vi "RT Driver VI.vi"(6 "Device Clock":string, 9 "Device Inputs FIFO":refnum<k33>, 10 "Device Outputs FIFO":refnum<k33>, 11 "Device Reference":T1 format="%.0x") -> ()   [LabVIEW 2025, in "Keithley-DAQ6510 Engine.lvlib"]
uses:
  Keithley-DAQ6510 Engine.lvlib
  <vilib>/NI VeriStand/Custom Device API/Custom Device Item Ref.ctl
  <vilib>/NI VeriStand/Custom Device API/Custom Device Channel Type.ctl
  RT_ctrl.ctl
  <vilib>/NI VeriStand/Custom Device API/Message Response (String).ctl
  <vilib>/NI VeriStand/Custom Device API/Message Response (Byte Array).ctl
  System Explorer/Sys_DAQ_Global.vi
  <vilib>/NI VeriStand/Custom Device API/Get Item Property (Variant).vi
  <vilib>/NI VeriStand/Custom Device API/Get Item Property (String).vi
  <vilib>/NI VeriStand/Custom Device API/Custom Device API.lvlib
  <vilib>/NI VeriStand/Custom Device Tools/Custom Device Utility Library/Custom Device Utility Library.lvlib
  System Explorer/Keithley-DAQ6510 System Explorer.lvlib
  <instrlib>/Keithley DMM6500 DAQ6500 Series/Keithley DMM6500 DAQ6500 Series.lvlib
panel:
  in  "Initialization Status Notifier":refnum<notifier>
  in  "Status Notifier":refnum<notifier>
  # "Custom Device Template\nv1.0"
  # "Use this template as a starting point for creating a custom device code module. The input controls shown here are specially named controls that the system will use to provide the device loop with data. The controls are not required for the device loop to run. For instance, if the device doesn't produce any output data, then you don't need the Device Outputs FIFO control. If you do use these controls, however, they need to have these exact names to be functional."
  # "The optional status notifier element is used to notify the RT engine of the last state of the custom device, and to indicate the device has completed execution. If this control is not used, a default No Error value is returned to the system when the device finishes execution.\n\nNote: This error state is not checked until the system shuts down. Use an output status channel to send more immediate status values to the system."
  # "This optional input can be used to send the VeriStand Engine the final status of the custom device initalization process. If this control exists on the custom device front panel, the VeriStand Engine will wait for a status update before starting up. If the custom device reports an error, that will abort the execution of the current configuration in the VeriStand Engine.\n\nThis control can be deleted if the custom device does not need to send the initialization status update."
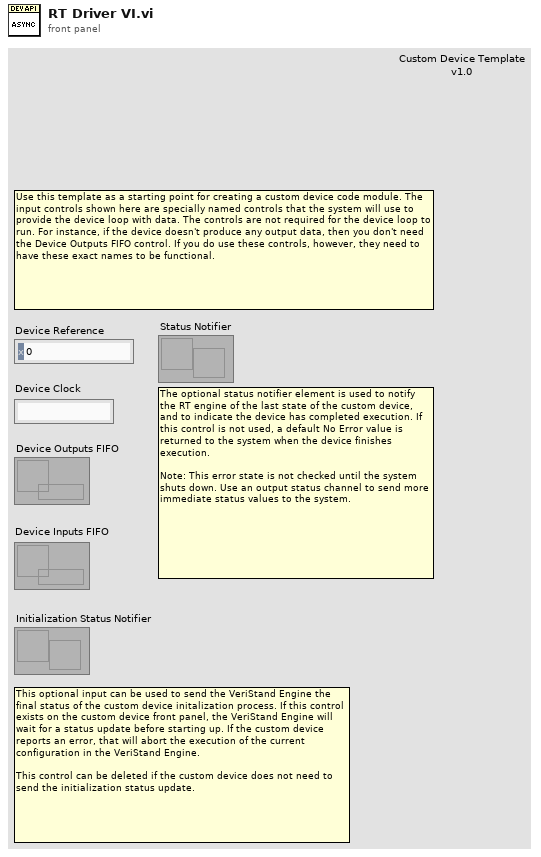
[diagram p1: front panel]
types:
  T1 = typedef "Custom Device API.lvlib/Custom Device Item Ref.ctl" = u64
  T2 = cluster{"Baud Rate":u32, "Flow Control":u16, "Parity":u16, "Stop Bits":u16, "Data Bits":u16}
  T3 = typedef "Keithley-DAQ6510 Engine.lvlib/RT_ctrl.ctl" = cluster{"Device Outputs FIFO":refnum<k33>, "Device Inputs FIFO":refnum<k33>, "Function":i32, "Pseudo Card":i32, "Slot":i32, "Channel_list":string, "Auto/Man":bool, "Manual Range":dbl, "VISA ":refnum<visa-resource-name>}
  T4 = typedef "Custom Device API.lvlib/Custom Device Channel Type.ctl" = enum16{"Input", "Output"}
  T5 = typedef "Custom Device API.lvlib/Custom Device Engine Event Ref.ctl" = refnum<event-registration>
  T6 = typedef "Custom Device API.lvlib/Message Response (String).ctl" = cluster{"Response":string, "Error":errorcluster}
  T7 = typedef "Custom Device API.lvlib/Message Response (Byte Array).ctl" = cluster{"Response":u8[], "Error":errorcluster}
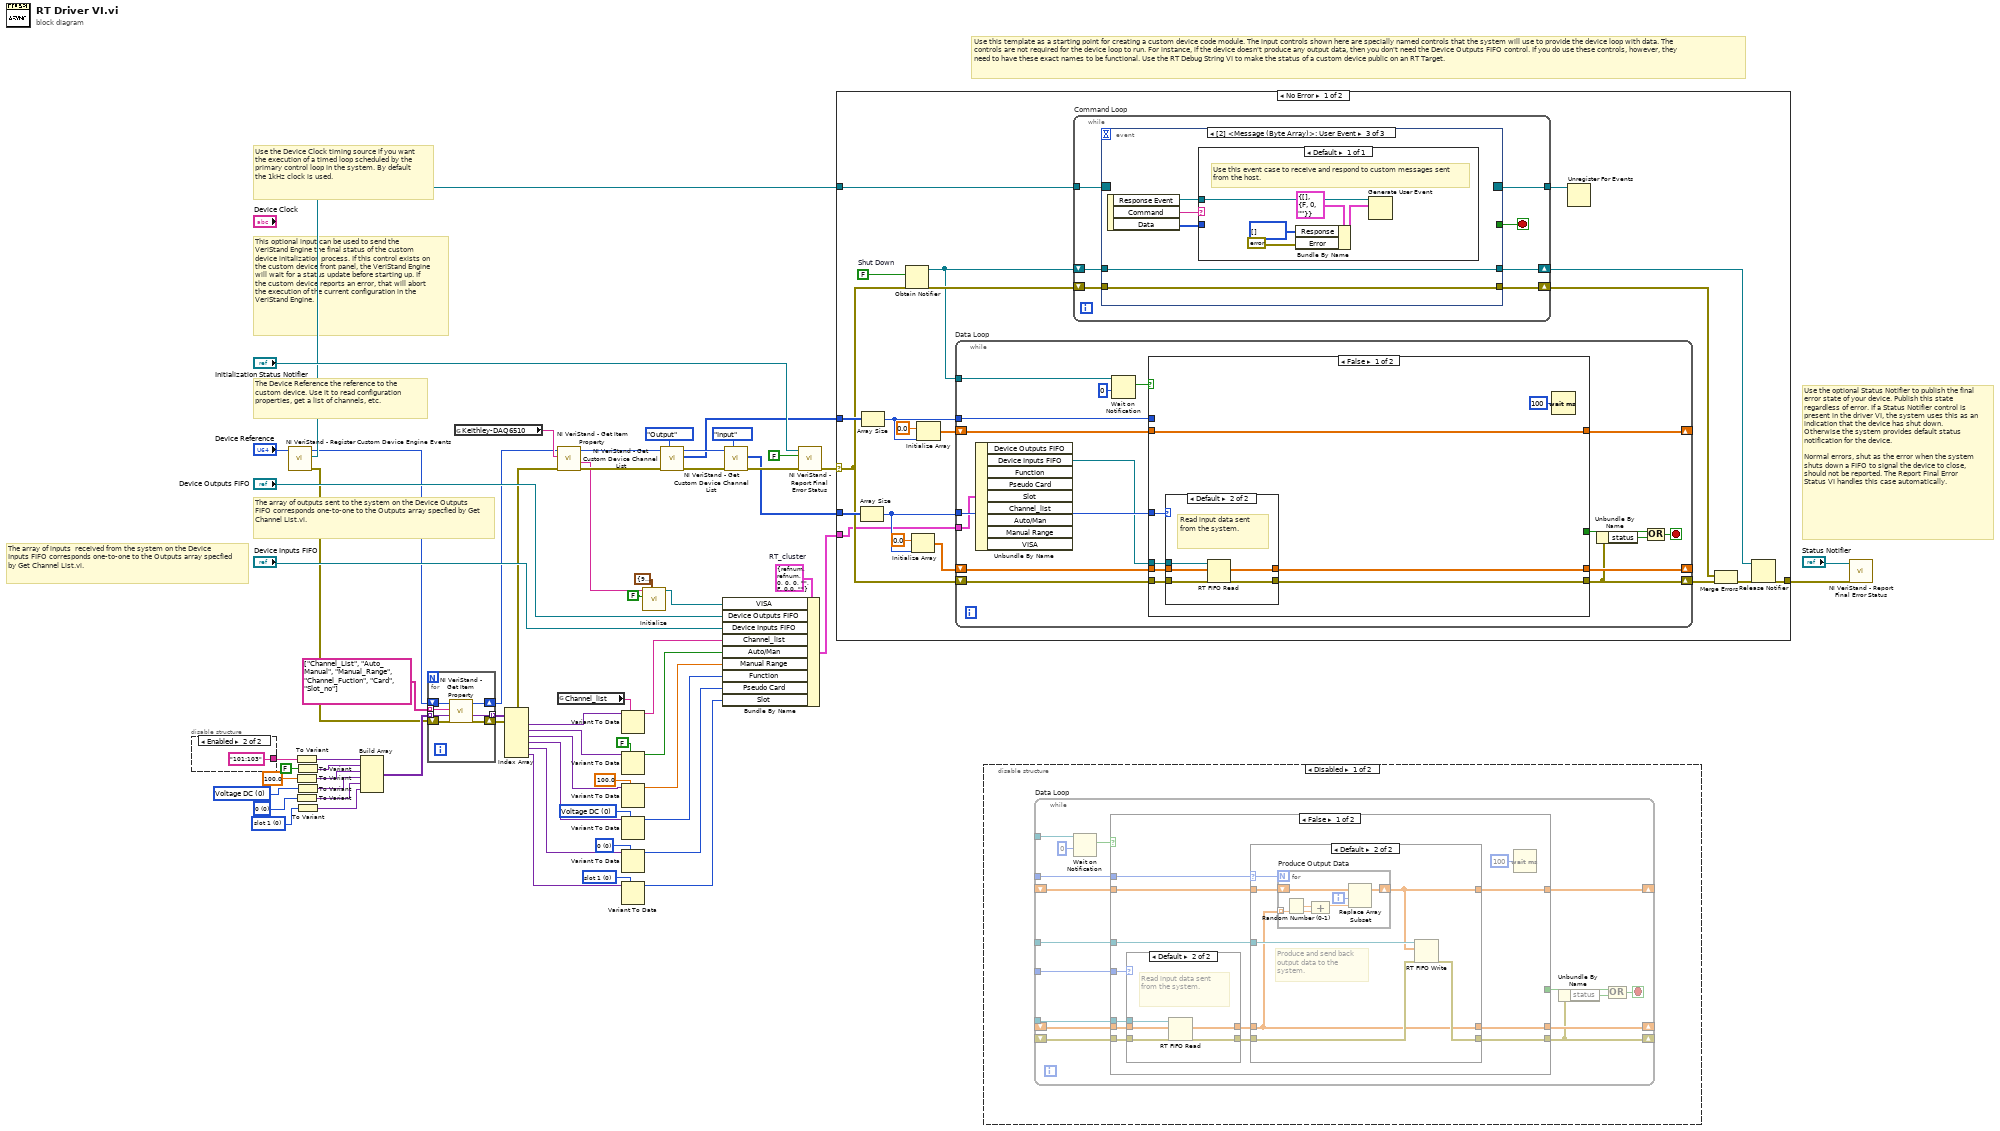
[diagram p0: block diagram]
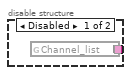
[diagram p2: hidden frame]
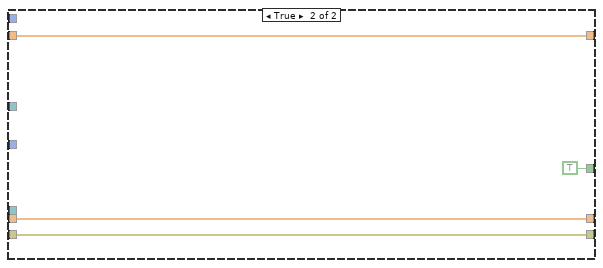
[diagram p5: hidden frame]
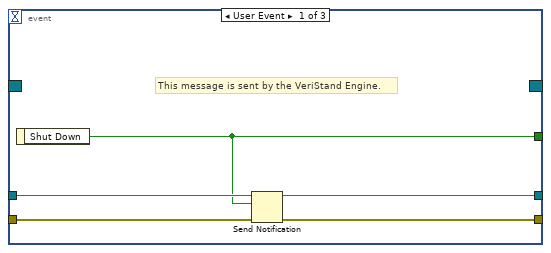
[diagram p7: hidden frame]
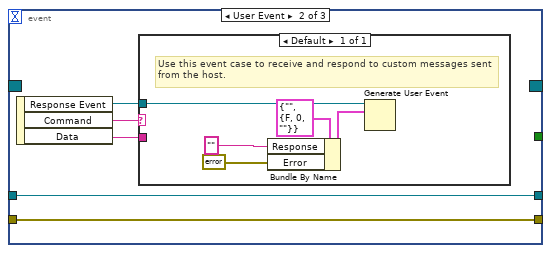
[diagram p8: hidden frame]
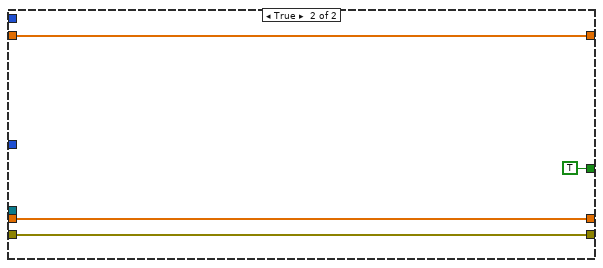
[diagram p10: hidden frame]
diagram:
  w34 = 0 items=["slot 1", "slot 2"] ("Slot Number (0: slot1)")
  w35 = 0 items=["0", "7700", "7701", "7702", "7703", "7705", "7706", "7707", "7708", "7709", "7710", "7711", "7712"] ("Pseudo Card (0:No pseudocard)")
  w36 = 0 items=["Voltage DC", "Voltage AC", "Current DC", "Current AC", "Resistance", "4-wire Resistance", "Diode", "Capacitance", "Temperature", "Continuity", "Frequency", "Period", "Voltage Ratio", "Digitize Voltage", "Digitize Current"] ("Function (0: Voltage DC)")
  w40 = 0 items=["slot 1", "slot 2"] ("Slot Number (0: slot1)")
  w41 = 0 items=["0", "7700", "7701", "7702", "7703", "7705", "7706", "7707", "7708", "7709", "7710", "7711", "7712"] ("Pseudo Card (0:No pseudocard)")
  w42 = 0 items=["Voltage DC", "Voltage AC", "Current DC", "Current AC", "Resistance", "4-wire Resistance", "Diode", "Capacitance", "Temperature", "Continuity", "Frequency", "Period", "Voltage Ratio", "Digitize Voltage", "Digitize Current"] ("Function (0: Voltage DC)")
  w48 = T3 {"Device Outputs FIFO"=refnum, "Device Inputs FIFO"=refnum, "Function"=0, "Pseudo Card"=0, "Slot"=0, "Channel_list"="", "Auto/Man"=FALSE, "Manual Range"=0.0, "VISA "=""}  # RT_cluster
  # "This optional input can be used to send the VeriStand Engine the final status of the custom device initalization process. If this control exists on the custom device front panel, the VeriStand Engine will wait for a status update before starting up. If the custom device reports an error, that will abort the execution of the current configuration in the VeriStand Engine."
  # "The array of inputs  received from the system on the Device Inputs FIFO corresponds one-to-one to the Outputs array specfied by Get Channel List.vi."
  # "Use the optional Status Notifier to publish the final error state of your device. Publish this state regardless of error. If a Status Notifier control is present in the driver VI, the system uses this as an indication that the device has shut down. Otherwise the system provides default status notification for the device.\n\nNormal errors, shut as the error when the system shuts down a FIFO to signal the device to close, should not be reported. The Report Final Error Status VI handles this case automatically."
  # "The array of outputs sent to the system on the Device Outputs FIFO corresponds one-to-one to the Outputs array specfied by Get Channel List.vi."
  # "The Device Reference the reference to the custom device. Use it to read configuration properties, get a list of channels, etc."
  # "Use the Device Clock timing source if you want the execution of a timed loop scheduled by the primary control loop in the system. By default the 1kHz clock is used."
  # "Use this template as a starting point for creating a custom device code module. The input controls shown here are specially named controls that the system will use to provide the device loop with data. The controls are not required for the device loop to run. For instance, if the device doesn't produce any output data, then you don't need the Device Outputs FIFO control. If you do use these controls, however, they need to have these exact names to be functional. Use the RT Debug String VI to make the status of a custom device public on an RT Target."
  n1 = disable-structure shown="Enabled" {
    disable-tunnel: [w63 "101:103" ("Channel_list")] -> w39
    frame Disabled {
      n2 = global read "Sys_DAQ_Global.vi" "Channel_list"() -> (w63:string)
    }
    frame Enabled {
    }
  }
  n3 = call <vilib>:"NI VeriStand - Register Custom Device Engine Events.vi"("Device Ref in"="Device Reference") -> ("error out"=w26:errorcluster, "Custom Device Engine Event Ref"=w53:T5, "Device Ref out"=w12:T1)  [unwired: 8 in]
  n4 = To Variant(anything=w39) -> (Variant=w33:variant)
  n5 = To Variant(anything=100.0) -> (Variant=w31:variant)
  n6 = To Variant(anything=w35) -> (Variant=w29:variant)
  n7 = To Variant(anything=FALSE) -> (Variant=w32:variant)
  n8 = To Variant(anything=w36) -> (Variant=w30:variant)
  n9 = To Variant(anything=w34) -> (Variant=w28:variant)
  n10 = Build Array(w33, w32, w31, w30, w29, w28) -> (w27:variant[])
  n11 = for {
    tunnel: w27 -> [w71] mode=indexing
    tunnel: string[] ["Channel_List", "Auto_Manual", "Manual_Range", "Channel_Fuction", "Card", "Slot_no"] ("Channel Name") -> [w69] mode=indexing
    shift-right: [w67] -> w7
    shift-left: w12 -> [w68]
    shift-right: [w66] -> w11
    shift-left: w26 -> [w70]
    tunnel: [w65] -> w24 mode=indexing
    n12 = call-poly <vilib>:"NI VeriStand - Get Item Property.vi"("error in (no error)"=w70, "Default Value"=w71, "Property Name"=w69, "Item Ref in"=w68) -> ("error out"=w66:errorcluster, "Value"=w65:variant, "Item Ref out"=w67:T1)  [unwired: 4 in, 1 out]
  }
  n13 = global read "Sys_DAQ_Global.vi" "Keithley-DAQ6510"() -> (w8:string)
  n14 = Index Array(array=w24) -> (element #1=w18:variant, element #2=w19:variant, element #3=w20:variant, element #4=w21:variant, element #5=w22:variant, element #6=w23:variant)  [unwired: 6 in]
  n15 = call-poly <vilib>:"NI VeriStand - Get Item Property.vi"("error in (no error)"=w11, "Property Name"=w8, "Item Ref in"=w7) -> ("error out"=w9:errorcluster, "Value"=w5:string, "Item Ref out"=w6:T1)  [unwired: 5 in, 1 out]
  n16 = global read "Sys_DAQ_Global.vi" "Channel_list"() -> (w45:string)
  n17 = Variant To Data(type=w45, Variant=w18) -> (data=w10:string)  [unwired: 1 in, 1 out]
  n18 = Variant To Data(type=FALSE, Variant=w19) -> (data=w17:bool)  [unwired: 1 in, 1 out]
  n19 = Variant To Data(type=100.0, Variant=w20) -> (data=w16:dbl)  [unwired: 1 in, 1 out]
  n20 = Variant To Data(type=w42, Variant=w21) -> (data=w15:i32)  [unwired: 1 in, 1 out]
  n21 = Variant To Data(type=w41, Variant=w22) -> (data=w14:i32)  [unwired: 1 in, 1 out]
  n22 = Variant To Data(type=w40, Variant=w23) -> (data=w13:i32)  [unwired: 1 in, 1 out]
  n23 = call <instrlib>:"Initialize.vi"("Serial Configuration"=T2 {"Baud Rate"=9600, "Flow Control"=0, "Parity"=0, "Stop Bits"=10, "Data Bits"=8}, "ID Query (True)"=FALSE, "VISA resource name"=w5) -> ("VISA resource name out"=w2:refnum<visa-resource-name>)  [unwired: 7 in, 1 out]
  n24 = call <vilib>:"NI VeriStand - Get Custom Device Channel List.vi"("Channel Type"=Custom_Device_Channel_Type."Output", "error in (no error)"=w9, "Device Ref in"=w6) -> ("error out"=w58:errorcluster, "Specified Channel Ref List"=w55:T1[], "Device Ref out"=w59:T1)  [unwired: 6 out]
  n25 = Bundle By Name(cluster=w48, "VISA"=w2, "Device Outputs FIFO"="Device Outputs FIFO", "Device Inputs FIFO"="Device Inputs FIFO", "Channel_list"=w10, "Auto/Man"=w17, "Manual Range"=w16, "Function"=w15, "Pseudo Card"=w14, "Slot"=w13) -> (w1:T3)
  n26 = call <vilib>:"NI VeriStand - Get Custom Device Channel List.vi"("Channel Type"=Custom_Device_Channel_Type."Input", "error in (no error)"=w58, "Device Ref in"=w59) -> ("error out"=w62:errorcluster, "Specified Channel Ref List"=w56:T1[])  [unwired: 7 out]
  n27 = call <vilib>:"NI VeriStand - Report Final Error Status.vi"("error in (no error)"=w62, "Filter FIFO & Shutdown Errors (T)"=FALSE ("Filter FIFO Errors (T)"), "Status Notifier"="Initialization Status Notifier") -> ("error out"=w50:errorcluster)  [unwired: 8 out]
  n28 = case shown="No Error" w50 {
    selector: w50 -> [w75 w159]
    tunnel: w56 -> [w85 _]
    tunnel: w55 -> [w84 _]
    tunnel: w53 -> [w82 _]
    tunnel: [w80 w159] -> w52
    tunnel: w1 -> [w72 _]
    frame No Error {
      w81 = FALSE  # Shut Down
      n29 = Array Size(array=w85) -> (size(s)=w83:i32)
      n30 = Array Size(array=w84) -> (size(s)=w86:i32)
      n31 = Obtain Notifier(notification data type=w81, error in (no error)=w75) -> (notifier out=w78:refnum<notifier>, error out=w91:errorcluster)  [unwired: 2 in, 1 out]
      n32 = Initialize Array(0.0 ("element"), w83) -> (w87:dbl[])
      n33 = Initialize Array(0.0 ("element"), w86) -> (w88:dbl[])
      n34 = while "Data Loop" {
        shift-right: [w137] -> _
        shift-left: w87 -> [w138]
        shift-right: [w131] -> w76
        shift-left: w75 -> [w139]
        shift-right: [w135] -> _
        shift-left: w88 -> [w136]
        tunnel: w86 -> [w134]
        tunnel: w83 -> [w133]
        tunnel: w78 -> [w130]
        tunnel: w72 -> [w125]
        stop <- w126 stop-if-true
        n35 = Unbundle By Name(w125) -> ("Device Inputs FIFO"=w124:refnum<k33>)  [unwired: 8 out]
        n36 = Wait on Notification(notifier=w130, timeout in ms (-1)=0) -> (notification=w129:bool)  [unwired: 2 in, 3 out]
        n37 = case shown="False" w129 {
          tunnel: w139 -> [w147 w157]
          tunnel: w138 -> [w146 w158]
          tunnel: [w141 w158] -> w137
          tunnel: w136 -> [w140 w156]
          tunnel: [w140 w156] -> w135
          tunnel: w124 -> [w145 _]
          tunnel: w134 -> [_ _]
          tunnel: w133 -> [w144 _]
          tunnel: [w142 w157] -> w131
          tunnel: [_ TRUE] -> w127
          frame False {
            n38 = case shown="Default" w144 {
              tunnel: w145 -> [_ w154]
              tunnel: w146 -> [w149 w153]
              tunnel: [w149 w152] -> w141
              tunnel: [w148 w151] -> w142
              tunnel: w147 -> [w148 w150]
              frame 0 {
                # "No inputs to read\nfrom system. Inputs FIFO not created in this case, so don't write to it."
              }
              frame Default {
                # "Read input data sent from the system."
                n39 = RT FIFO Read(0:w154, 1:w153, 3:w150) -> (9:w152:dbl[], 11:w151:errorcluster)  [unwired: 4 out]
              }
            }
            n40 = Wait (ms)(milliseconds to wait=u32 100) -> ()  [unwired: 1 out]
          }
          frame True {
          }
        }
        n41 = Unbundle By Name(w131) -> ("status"=w128:bool)
        n42 = Compound Arithmetic op=OR(w127, w128) -> (w126:bool)
      }
      n43 = while "Command Loop" {
        tunnel: w82 -> [w98]
        tunnel: [w97] -> w79
        shift-right: [w94] -> w77
        shift-left: w78 -> [w95]
        shift-right: [w92] -> w73
        shift-left: w91 -> [w93]
        stop <- w96 stop-if-true
        n44 = event shown="[2] <Message (Byte Array)>: User Event" {
          selector: w98 -> [_ _ _]
          dyn-events: [_ _ _] -> w97
          timeout: _ -> [_ _ _]
          tunnel: [w101 _ _] -> w96
          tunnel: w95 -> [w102 w106 w116]
          tunnel: [w103 w106 w116] -> w94
          tunnel: w93 -> [w100 w104 w114]
          tunnel: [w99 w104 w114] -> w92
          event User Event {
            # "This message is sent by the VeriStand Engine."
            n45 = event-data() -> ("Shut Down"=w101:bool)  [unwired: 1 in]
            n46 = Send Notification(notification=w101, notifier=w102, error in (no error)=w100) -> (notifier out=w103:refnum<notifier>, error out=w99:errorcluster)
          }
          event User Event {
            n47 = event-data() -> ("Response Event"=w105:refnum<user-event>, "Command"=w108:string, "Data"=w107:string)  [unwired: 1 in]
            n48 = case shown="Default" w108 {
              tunnel: w107 -> [_]
              tunnel: w105 -> [w113]
              frame Default {
                # "Use this event case to receive and respond to custom messages sent from the host."
                n49 = Bundle By Name(cluster=T6 {"Response"="", "Error"={"status"=FALSE, "code"=0, "source"=""}} ("event data"), "Response"="", "Error"=errorcluster {"status"=FALSE, "code"=0, "source"=""}) -> (w111:T6)
                n50 = Generate User Event(user event=w113, event data cluster=w111) -> ()  [unwired: 2 in, 2 out]
              }
            }
          }
          event User Event {
            n51 = event-data() -> ("Response Event"=w115:refnum<user-event>, "Command"=w118:string, "Data"=w117:u8[])  [unwired: 1 in]
            n52 = case shown="Default" w118 {
              tunnel: w117 -> [_]
              tunnel: w115 -> [w123]
              frame Default {
                # "Use this event case to receive and respond to custom messages sent from the host."
                n53 = Bundle By Name(cluster=T7 {"Response"=[], "Error"={"status"=FALSE, "code"=0, "source"=""}} ("event data"), "Response"=u8[] [], "Error"=errorcluster {"status"=FALSE, "code"=0, "source"=""}) -> (w120:T7)
                n54 = Generate User Event(user event=w123, event data cluster=w120) -> ()  [unwired: 2 in, 2 out]
              }
            }
          }
        }
      }
      n55 = Unregister For Events(event registration refnum=w79) -> ()  [unwired: 1 in, 1 out]
      n56 = Merge Errors(w73, w76) -> (w74:errorcluster)
      n57 = Release Notifier(notifier=w77, error in (no error)=w74) -> (error out=w80:errorcluster)  [unwired: 1 in, 2 out]
    }
    frame Error {
    }
  }
  n58 = disable-structure shown="Disabled" {
    frame Disabled {
      n59 = while "Data Loop" {
        shift-right: [w173] -> _
        shift-left: _ -> [w174]
        shift-right: [w165] -> _
        shift-left: _ -> [w175]
        shift-right: [w171] -> _
        shift-left: _ -> [w172]
        tunnel: _ -> [w168]
        tunnel: _ -> [w170]
        tunnel: _ -> [w169]
        tunnel: _ -> [w167]
        tunnel: _ -> [w164]
        stop <- w160 stop-if-true
        n60 = Wait on Notification(notifier=w164, timeout in ms (-1)=0) -> (notification=w163:bool)  [unwired: 2 in, 3 out]
        n61 = case shown="False" w163 {
          tunnel: w175 -> [w188 w214]
          tunnel: w174 -> [w187 w215]
          tunnel: [w186 w215] -> w173
          tunnel: w172 -> [w185 w213]
          tunnel: [w184 w213] -> w171
          tunnel: w170 -> [w183 _]
          tunnel: w169 -> [w182 _]
          tunnel: w168 -> [w181 _]
          tunnel: w167 -> [w180 _]
          tunnel: [w177 w214] -> w165
          tunnel: [_ TRUE] -> w161
          frame False {
            n62 = case shown="Default" w180 {
              tunnel: w182 -> [_ w211]
              tunnel: w187 -> [w206 w210]
              tunnel: [w206 w209] -> w179
              tunnel: [w205 w208] -> w178
              tunnel: w188 -> [w205 w207]
              frame 0 {
                # "No inputs to read\nfrom system. Inputs FIFO not created in this case, so don't write to it."
              }
              frame Default {
                # "Read input data sent from the system."
                n63 = RT FIFO Read(0:w211, 1:w210, 3:w207) -> (9:w209:dbl[], 11:w208:errorcluster)  [unwired: 4 out]
              }
            }
            n64 = case shown="Default" w181 {
              selector: w181 -> [_ w192]
              tunnel: w183 -> [_ w198]
              tunnel: w185 -> [w191 w197]
              tunnel: w179 -> [w190 w193]
              tunnel: w178 -> [w189 w196]
              tunnel: [w189 w195] -> w177
              tunnel: [w191 w194] -> w184
              tunnel: [w190 w193] -> w186
              frame 0 {
                # "No outputs to write to system. The Device Outputs FIFO is never created in this case, so don't write to it."
              }
              frame Default {
                # "Produce and send back output data to the system."
                n65 = for "Produce Output Data" {
                  N: w192 -> [_]
                  shift-right: [w203] -> w194
                  shift-left: w197 -> [w204]
                  tunnel: w193 -> [w199] mode=indexing
                  i -> [w202]
                  n66 = Random Number (0-1)() -> (number: 0 to 1=w201:dbl)
                  n67 = Compound Arithmetic op=ADD(w201, w199) -> (w200:dbl)
                  n68 = Replace Array Subset(array=w204, new element=w200, index=w202) -> (w203:dbl[])
                }
                n69 = RT FIFO Write(0:w198, 1:w194, 3:w196) -> (11:w195:errorcluster)  [unwired: 1 in, 4 out]
              }
            }
            n70 = Wait (ms)(milliseconds to wait=u32 100) -> ()  [unwired: 1 out]
          }
          frame True {
          }
        }
        n71 = Unbundle By Name(w165) -> ("status"=w162:bool)
        n72 = Compound Arithmetic op=OR(w161, w162) -> (w160:bool)
      }
    }
    frame Enabled {
    }
  }
  n73 = call <vilib>:"NI VeriStand - Report Final Error Status.vi"("error in (no error)"=w52, "Status Notifier"="Status Notifier") -> ()  [unwired: 1 in, 9 out]
